vi "Save Edited Entry.vi"(6 "Project Store in":refnum<class "Project Store.lvclass">, 7 "Time Entry Store in":refnum<class "Time Entry Store.lvclass">, 8 "error in":errorcluster, 10 "Edited Entry":T1, 11 "Original Entry":T1) -> (0 "error out":errorcluster, 3 "Saved Entry":T1, 5 "Time Entry Store out":refnum<class "Time Entry Store.lvclass">)   [LabVIEW 2026]
doc: "Saves a time entry after the user has edited it. Month files are chosen by the UTC month of Start Time, so when the edit moves Start Time into another UTC month the entry is first deleted from the original month file (with the ORIGINAL Start Time) and then saved into the new one. Otherwise it is just saved, which overwrites the row with the same ID.\n\nInputs: Original Entry (as it was read); Edited Entry (same ID, new values); Time Entry Store in; Project Store in (optional, supplies the name labels written to the file); error in.\nOutputs: Saved Entry; Time Entry Store out; error out.\n\nGenerated by: Claude"
uses:
  Storage/Rows/Time Entry.ctl
  Storage/Time Entry Store/Time Entry Store.lvclass
  Storage/Project Store/Project Store.lvclass
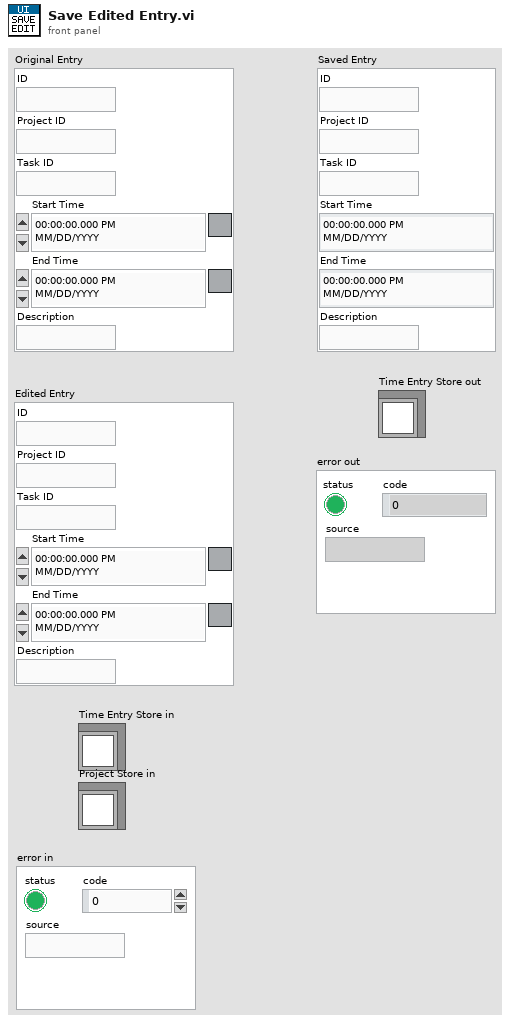
[diagram p1: front panel]
types:
  T1 = typedef "Time Entry.ctl" = cluster{"ID":string, "Project ID":string, "Task ID":string, "Start Time":timestamp, "End Time":timestamp, "Description":string}
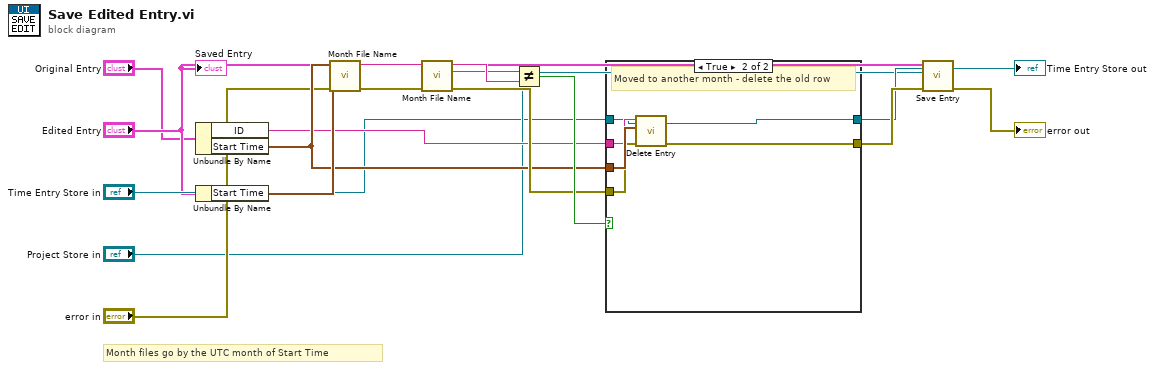
[diagram p0: block diagram]
diagram:
  # "Month files go by the UTC month of Start Time"
  n1 = Unbundle By Name("Original Entry") -> ("ID"=w8:string, "Start Time"=w9:timestamp)
  n2 = Unbundle By Name("Edited Entry") -> ("Start Time"=w10:timestamp)
  n3 = call "Month File Name.vi"("error in (no error)"="error in", "Start Time"=w9) -> ("error out"=w12:errorcluster, "File Name"=w11:string)  [unwired: 8 in]
  n4 = call "Month File Name.vi"("error in (no error)"=w12, "Start Time"=w10) -> ("error out"=w14:errorcluster, "File Name"=w13:string)  [unwired: 8 in]
  n5 = Not Equal?(x=w11, y=w13) -> (x != y?=w15:bool)
  n6 = case shown="True" w15 {
    tunnel: "Time Entry Store in" -> [w18 w20]
    tunnel: w8 -> [_ w22]
    tunnel: w9 -> [_ w23]
    tunnel: [w18 w24] -> w16
    tunnel: w14 -> [w19 w21]
    tunnel: [w19 w25] -> w17
    frame False {
      # "Same month file"
    }
    frame True {
      # "Moved to another month - delete the old row"
      n7 = call-dynamic "Delete Entry.vi"("Time Entry Store in"=w20, "error in (no error)"=w21, "Start Time"=w23, "ID"=w22) -> ("error out"=w25:errorcluster, "Time Entry Store out"=w24:refnum<class "Time Entry Store.lvclass">)  [unwired: 5 in, 1 out]
    }
  }
  n8 = call-dynamic "Save Entry.vi"("Time Entry Store in"=w16, "error in (no error)"=w17, "Project Store"="Project Store in", "Time Entry"="Edited Entry") -> ("error out"=→"error out":errorcluster, "Time Entry Store out"=→"Time Entry Store out":refnum<class "Time Entry Store.lvclass">)  [unwired: 6 in]
  "Saved Entry" <- "Edited Entry"
